vi "Compare LabVIEW File.vi"(6 "Interactive?":bool, 8 "error in":errorcluster, 10 "Results Directory":path, 11 "File Info in":T1) -> (0 "error out":errorcluster, 3 "File Info out":T1)   [LabVIEW 2020, in "Peer Review.lvclass"]
uses:
  Peer Review.lvclass
  TypeDefs/File Info.ctl
  TypeDefs/File State.ctl
  TypeDefs/VI Type.ctl
  Peer Review.lvclass/Peer Review.ctl
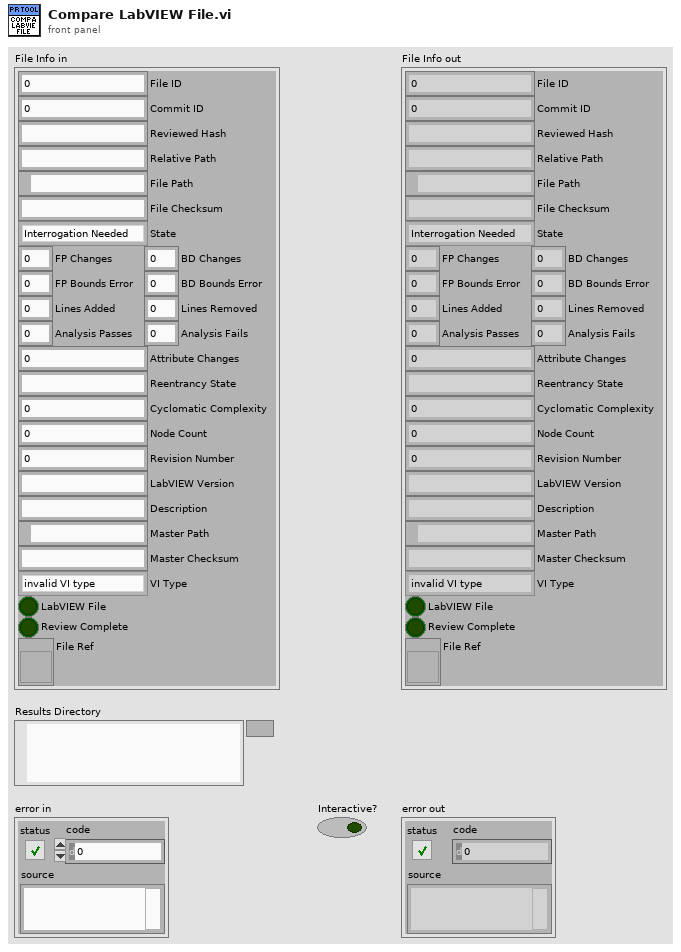
[diagram p1: front panel]
types:
  T1 = typedef "Peer Review.lvclass/File Info.ctl" = cluster{"File ID":i32, "Commit ID":i32, "Reviewed Hash":string, "Relative Path":string, "File Path":path, "File Checksum":string, "State":T2, "FP Changes":i32, "BD Changes":i32, "FP Bounds Error":dbl, "BD Bounds Error":dbl, "Lines Added":i32, "Lines Removed":i32, "Analysis Passes":i32, "Analysis Fails":i32, "Attribute Changes":i32, "Reentrancy State":string, "Cyclomatic Complexity":i32, "Node Count":i32, "Revision Number":u32, "LabVIEW Version":string, "Description":string, "Master Path":path, "Master Checksum":string, "VI Type":T3, "LabVIEW File":bool, "Review Complete":bool, "File Ref":refnum<vi>}
  T2 = typedef "Peer Review.lvclass/File State.ctl" = enum16{"Interrogation Needed", "Modified", "Deleted", "Added", "Matches Previous", "No Changes", "Moved"}
  T3 = typedef "Peer Review.lvclass/VI Type.ctl" = enum32{"invalid VI type", "Standard VI", "Control VI", "Global VI", "Polymorphic VI", "Configuration VI", "SubSystem", "Facade VI", "Method VI", "Statechart Diagram VI"}
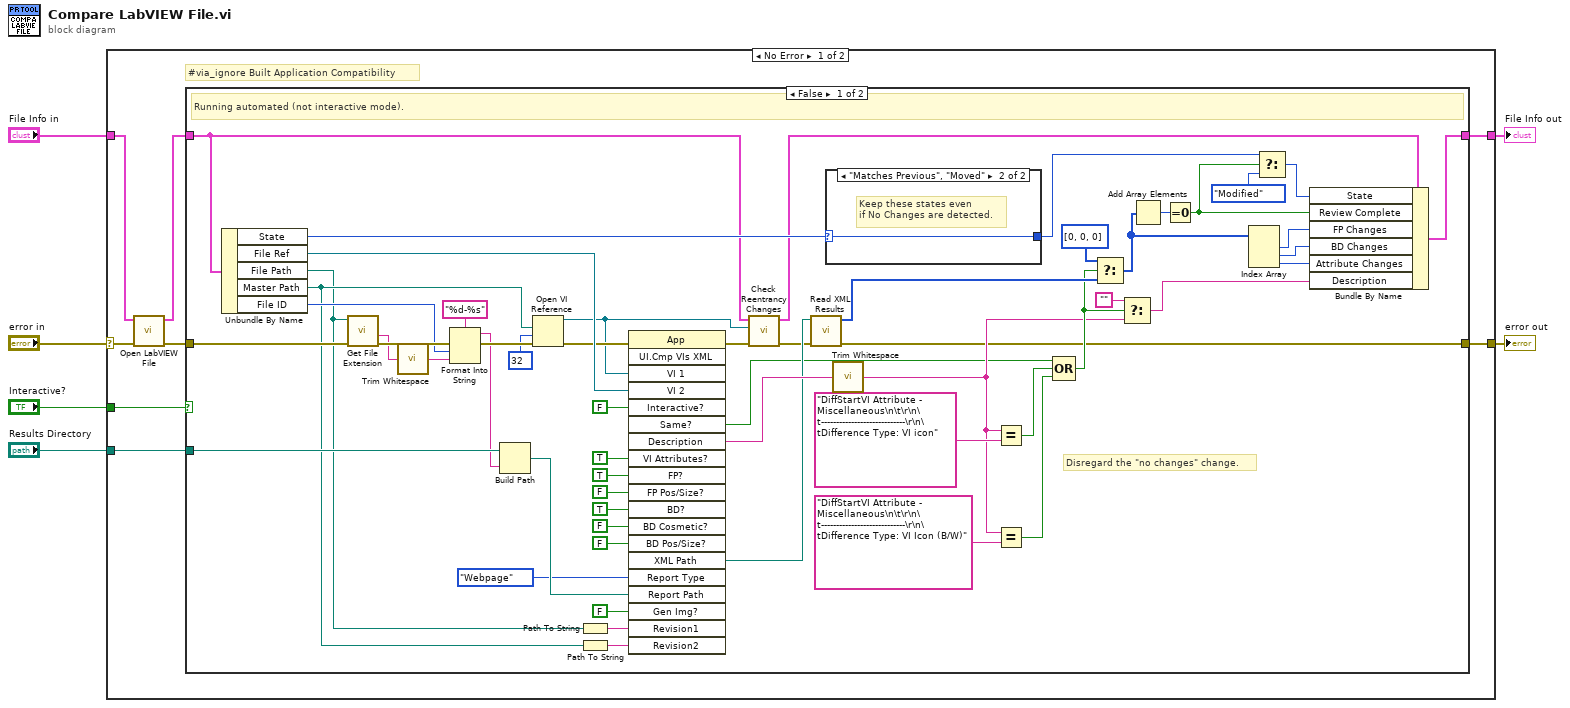
[diagram p0: block diagram]
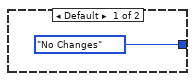
[diagram p2: hidden frame]
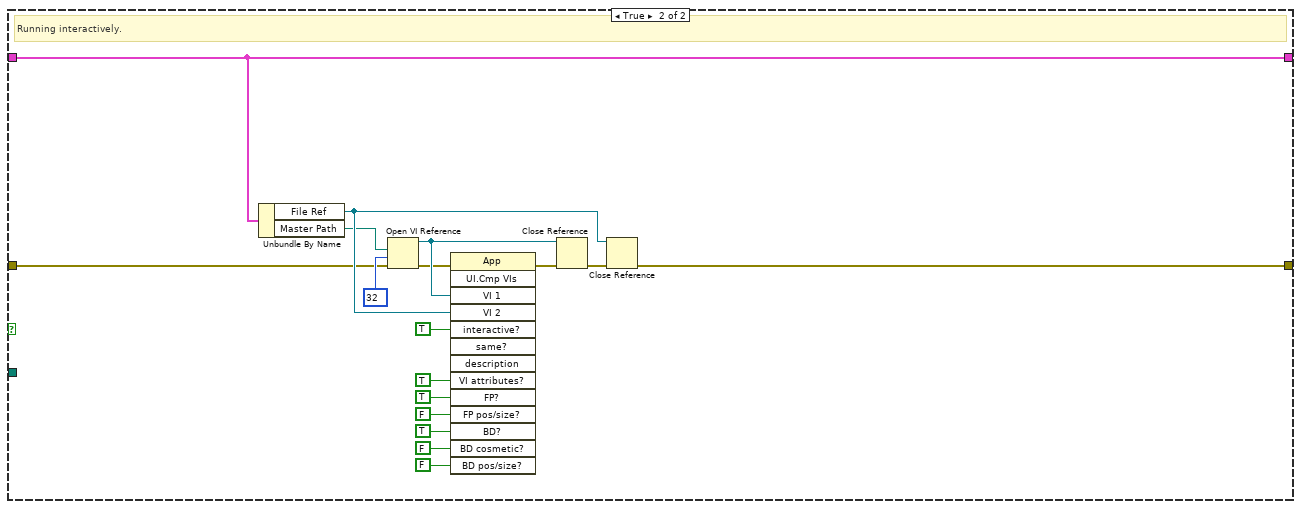
[diagram p3: hidden frame]
diagram:
  n1 = case shown="No Error" "error in" {
    selector: "error in" -> [w10 w91]
    tunnel: "File Info in" -> [w7 w90]
    tunnel: "Interactive?" -> [w11 _]
    tunnel: [w14 w90] -> w4
    tunnel: [w13 w91] -> w3
    tunnel: "Results Directory" -> [w12 _]
    frame No Error {
      # "#via_ignore Built Application Compatibility"
      n2 = call "Open LabVIEW File.vi"("error in"=w10, "File Info in"=w7) -> ("error out"=w9:errorcluster, "File Info out"=w8:T1)  [unwired: 8 in]
      n3 = case shown="False" w11 {
        tunnel: [w20 w76] -> w14
        tunnel: [w21 w78] -> w13
        tunnel: w12 -> [w68 _]
        tunnel: w9 -> [w65 w74]
        tunnel: w8 -> [w18 w76]
        frame False {
          # "Disregard the \"no changes\" change."
          # "Running automated (not interactive mode)."
          n4 = Unbundle By Name(w18) -> ("State"=w54:T2, "File Ref"=w44:refnum<vi>, "File Path"=w46:path, "Master Path"=w48:path, "File ID"=w52:i32)
          n5 = call <vilib>:"Get File Extension.vi"("error in (no error)"=w65, "file"=w46) -> ("error out"=w66:errorcluster, "filename without extension"=w51:string)  [unwired: 5 in, 3 out]
          n6 = call <vilib>:"Trim Whitespace.vi"("string"=w51) -> ("trimmed string"=w50:string)  [unwired: 1 in]
          n7 = Format Into String(format string="%d-%s", error in=w66, w52, w50) -> (resulting string=w49:string, error out=w64:errorcluster)  [unwired: 1 in]
          n8 = Build Path(base path=w68, name or relative path=w49) -> (appended path=w67:path)
          n9 = Open VI Reference(vi path=w48, options=32, error in (no error)=w64) -> (vi reference=w17:refnum<vi>, error out=w43:errorcluster)  [unwired: 1 in, 2 out]
          n10 = Path To String(path=w46) -> (string=w62:string)
          n11 = Path To String(path=w48) -> (string=w63:string)
          n12 = invoke on="Invoke Node" class="App" method="UI.Cmp VIs XML"(error in=w43, "VI 1"=w17, "VI 2"=w44, "Interactive?"=FALSE, "VI Attributes?"=TRUE, "FP?"=TRUE, "FP Pos/Size?"=FALSE, "BD?"=TRUE, "BD Cosmetic?"=FALSE, "BD Pos/Size?"=FALSE, "Report Type"=enum32{"None", "Webpage", "Text", "MS Word"}."Webpage", "Report Path"=w67, "Gen Img?"=FALSE, "Revision1"=w62, "Revision2"=w63) -> (error out=w45:errorcluster, "Same?"=w15:bool, "Description"=w70:string, "XML Path"=w47:path)  [unwired: 5 in, 16 out]
          n13 = call "Check Reentrancy Changes.vi"("error in"=w45, "Master VI Ref"=w17, "File Info in"=w18) -> ("error out"=w23:errorcluster, "File Info out"=w19:T1)  [unwired: 7 in]
          n14 = call "Read XML Results.vi"("error in"=w23, "XML Path"=w47) -> ("error out"=w21:errorcluster, "Changes"=w28:i32[])  [unwired: 8 in]
          n15 = case shown="\"Matches Previous\", \"Moved\"" w54 {
            selector: w54 -> [_ w72]
            tunnel: [File_State."No Changes" ("f") w72] -> w22
            frame Default {
            }
            frame "Matches Previous", "Moved" {
              # "Keep these states even\nif No Changes are detected."
            }
          }
          n16 = call <vilib>:"Trim Whitespace.vi"("string"=w70) -> ("trimmed string"=w24:string)  [unwired: 1 in]
          n17 = Equal?(x=w24, y="DiffStartVI Attribute - Miscellaneous\n\t\r\n\t----------------------------\r\n\tDifference Type: VI icon" ("Display")) -> (x = y?=w33:bool)
          n18 = Equal?(x=w24, y="DiffStartVI Attribute - Miscellaneous\n\t\r\n\t----------------------------\r\n\tDifference Type: VI Icon (B/W)" ("Description")) -> (x = y?=w34:bool)
          n19 = Compound Arithmetic op=OR(w15, w33, w34) -> (w25:bool)
          n20 = Select(t=i32[] [0, 0, 0] ("Changes"), s=w25, f=w28) -> (s? t:f=w26:i32[])
          n21 = Select(t="" ("Empty String Constant"), s=w25, f=w24) -> (s? t:f=w27:string)
          n22 = Add Array Elements(numeric array=w26) -> (sum=w40:i32)
          n23 = Equal To 0?(x=w40) -> (x = 0?=w31:bool)
          n24 = Index Array(array=w26) -> (element #1=w37:i32, element #2=w38:i32, element #3=w39:i32)  [unwired: 3 in]
          n25 = Select(t=w22, s=w31, f=File_State."Modified") -> (s? t:f=w32:T2)
          n26 = Bundle By Name(cluster=w19, "State"=w32, "Review Complete"=w31, "FP Changes"=w37, "BD Changes"=w38, "Attribute Changes"=w39, "Description"=w27) -> (w20:T1)
        }
        frame True {
          # "Running interactively."
          n27 = Unbundle By Name(w76) -> ("File Ref"=w75:refnum<vi>, "Master Path"=w73:path)
          n28 = Open VI Reference(vi path=w73, options=32, error in (no error)=w74) -> (vi reference=w82:refnum<vi>, error out=w80:errorcluster)  [unwired: 1 in, 2 out]
          n29 = invoke on="Invoke Node" class="App" method="UI.Cmp VIs"(error in=w80, "VI 1"=w82, "VI 2"=w75, "interactive?"=TRUE ("Interactive?"), "VI attributes?"=TRUE ("VI Attributes?"), "FP?"=TRUE, "FP pos/size?"=FALSE ("FP Pos/Size?"), "BD?"=TRUE, "BD cosmetic?"=FALSE ("BD Cosmetic?"), "BD pos/size?"=FALSE ("BD Pos/Size?")) -> (error out=w83:errorcluster)  [unwired: 4 in, 13 out]
          n30 = Close Reference(reference=w82, error in (no error)=w83) -> (error out=w79:errorcluster)
          n31 = Close Reference(reference=w75, error in (no error)=w79) -> (error out=w78:errorcluster)
        }
      }
    }
    frame Error {
    }
  }
  "File Info out" <- w4
  "error out" <- w3
